vi "Base edit mode.vi"(8 "error in":errorcluster caption="エラー入力（エラーなし）") -> (0 "error out":errorcluster caption="エラー出力", 3 "Base All Composition_out":T1(array[cluster]))   [LabVIEW 2018]
panel:
  in  "R_index":i32
  out "result_number":string
  out "path":path
  in  "N_element":string
  out "filenames":string[](array[string])
  out "stripped path":path
  out "element":string
  in  "insert index":i32
  in  "Base All Composition_edit":T1(array[cluster])
  in  "Base Insert":bool
  in  "New Recipe Creat":bool
  in  "stop":bool
  in  "Edit_index":i32
  in  "Item":T2
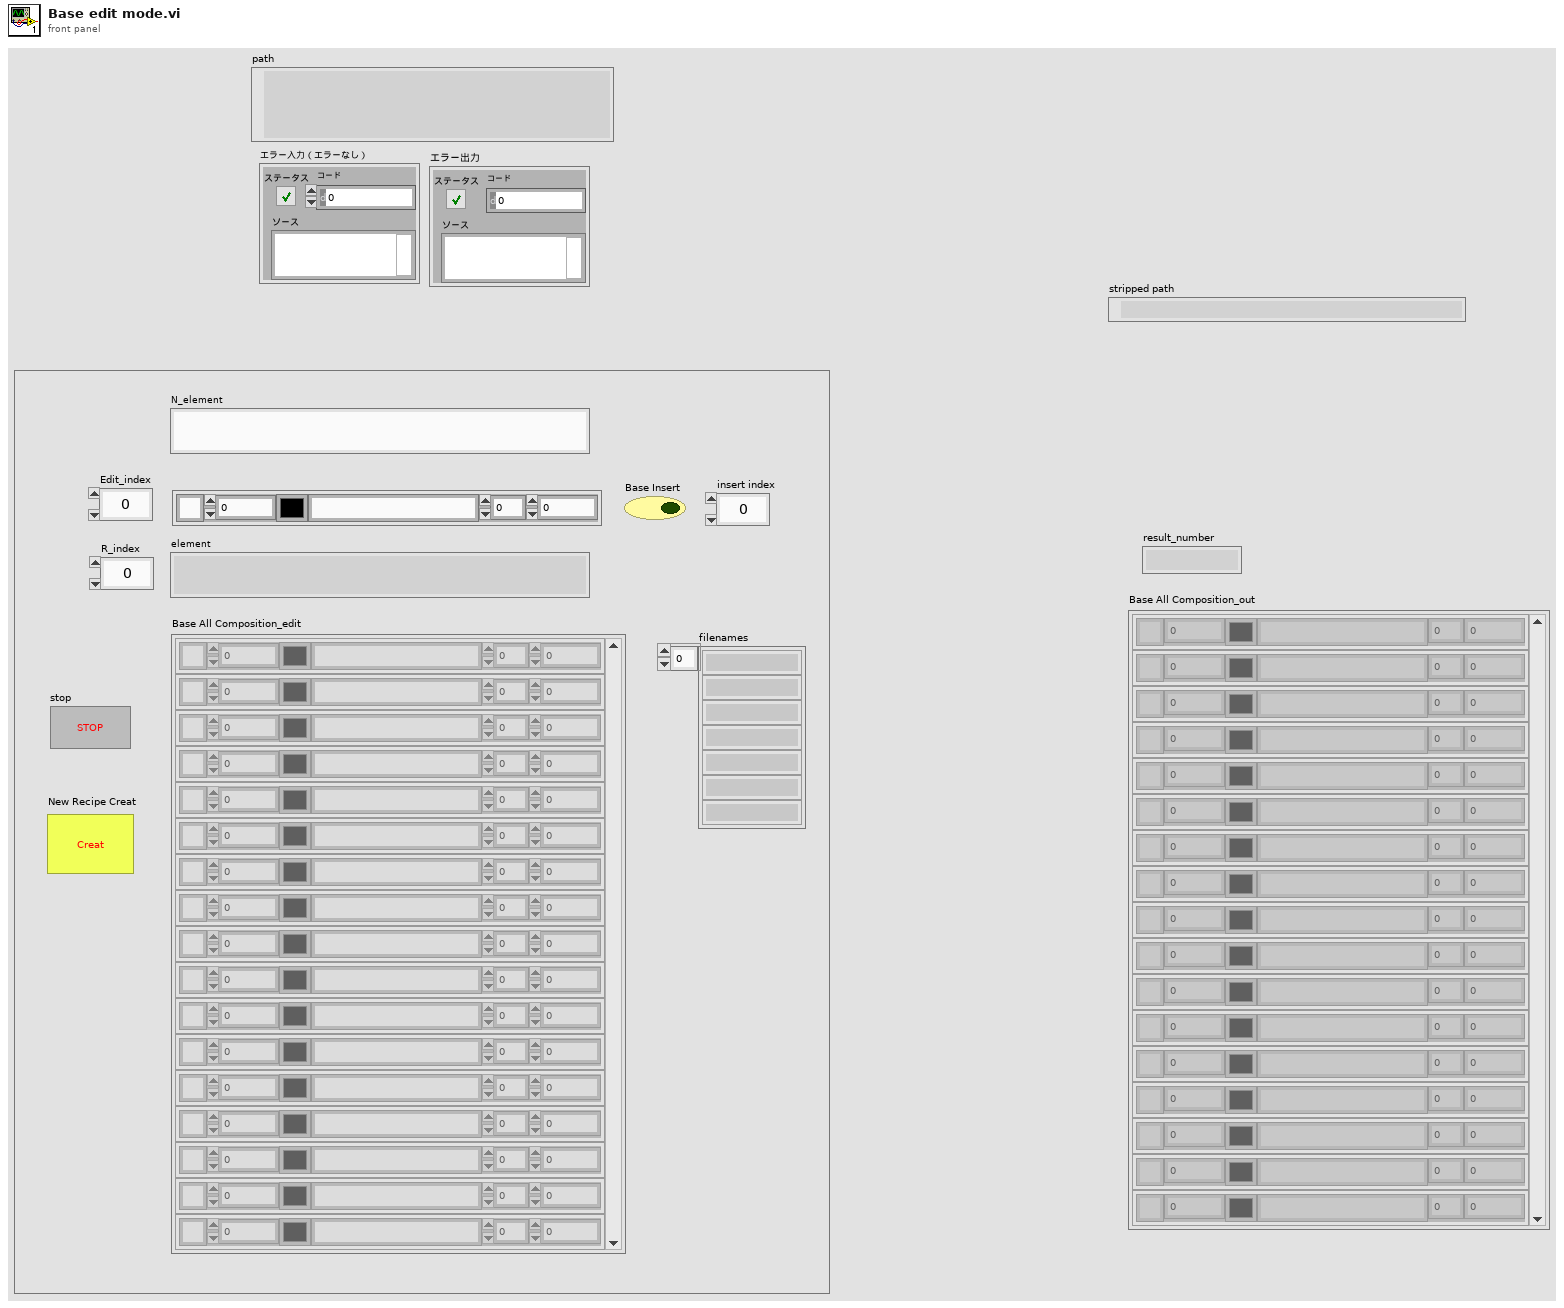
[diagram p1: front panel]
types:
  T1 = cluster{"Name":string, "Value":dbl, "Color":u32, "Name 2":string, "Value 2":dbl, "Value 3":dbl}[]
  T2 = cluster{"Name":string, "Value":dbl, "Color":u32, "Name 2":string, "Value 2":dbl, "Value 3":dbl}
  T3 = enum16{"open", "replace", "create", "open or create", "replace or create", "replace or create with confirmation"}
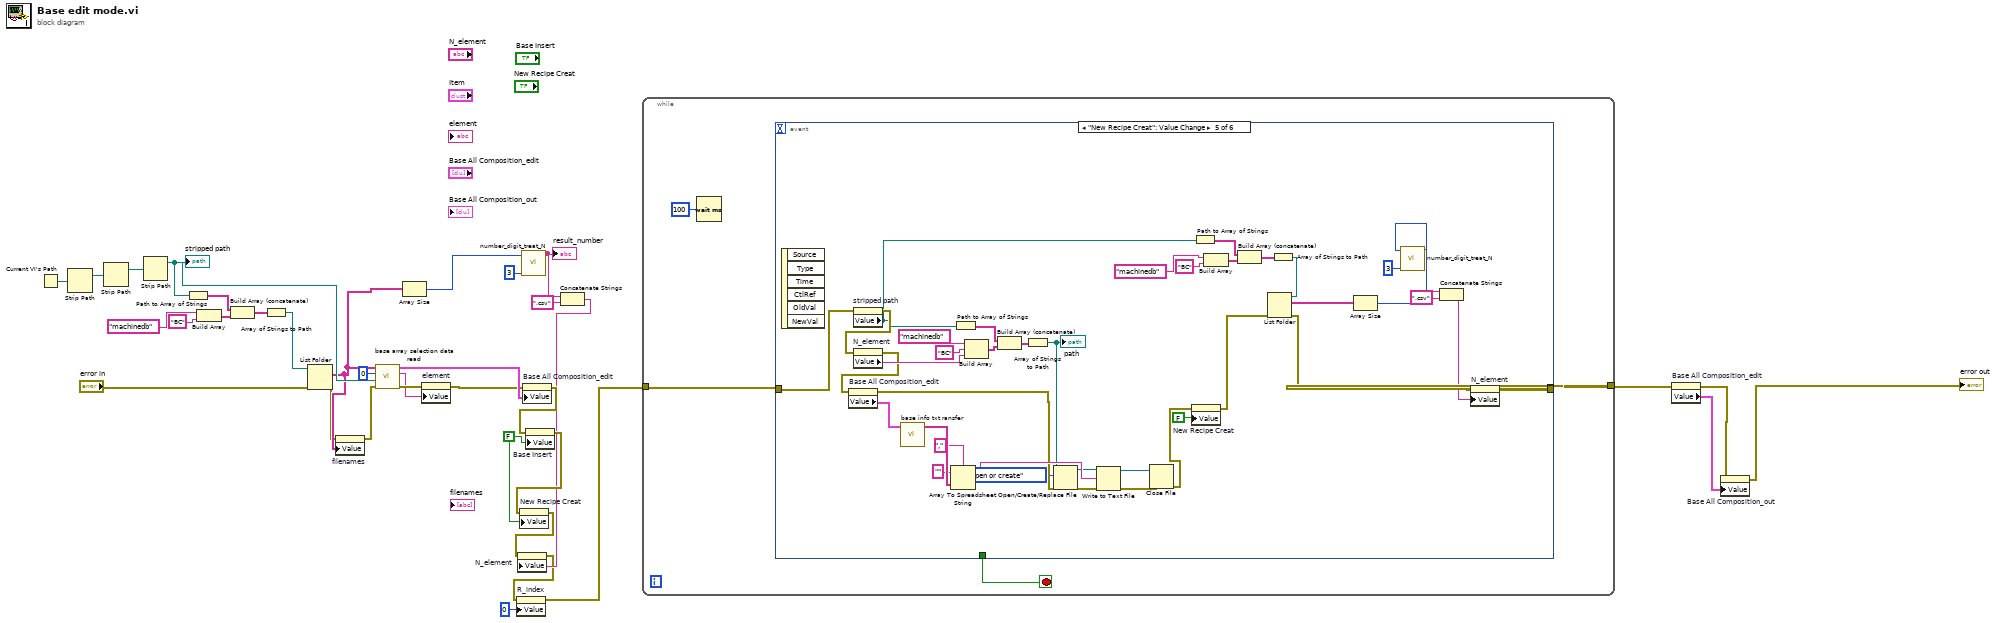
[diagram p0: block diagram]
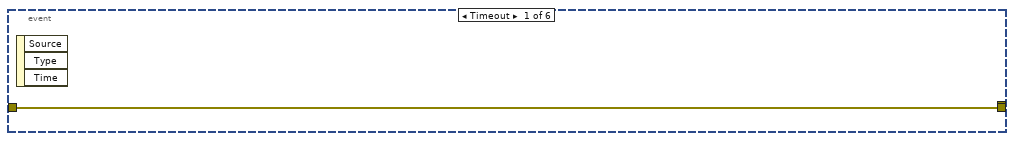
[diagram p2: hidden frame]
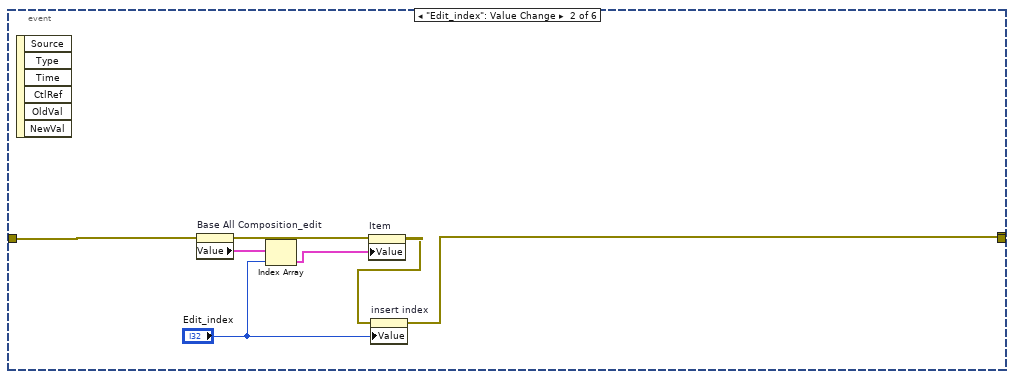
[diagram p3: hidden frame]
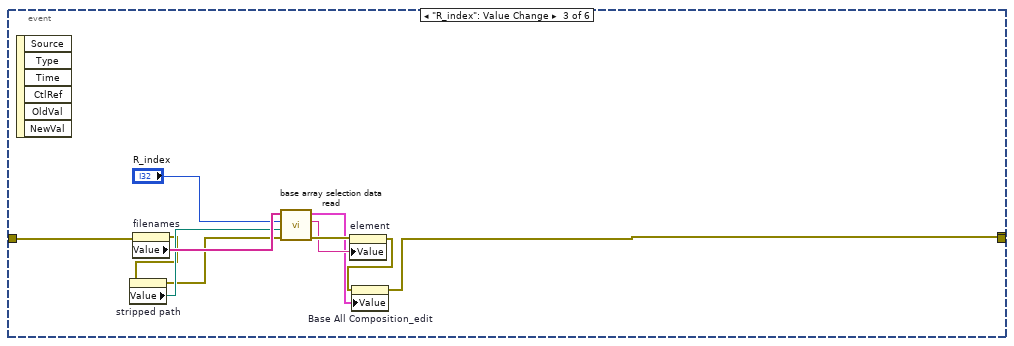
[diagram p4: hidden frame]
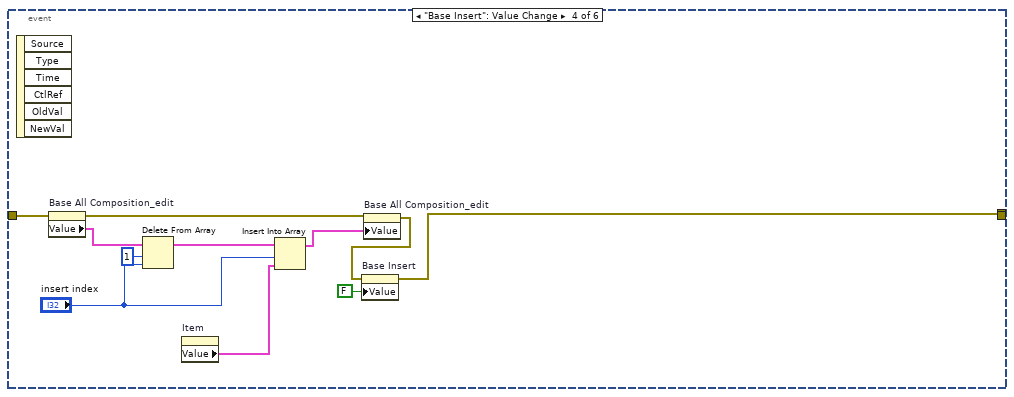
[diagram p5: hidden frame]
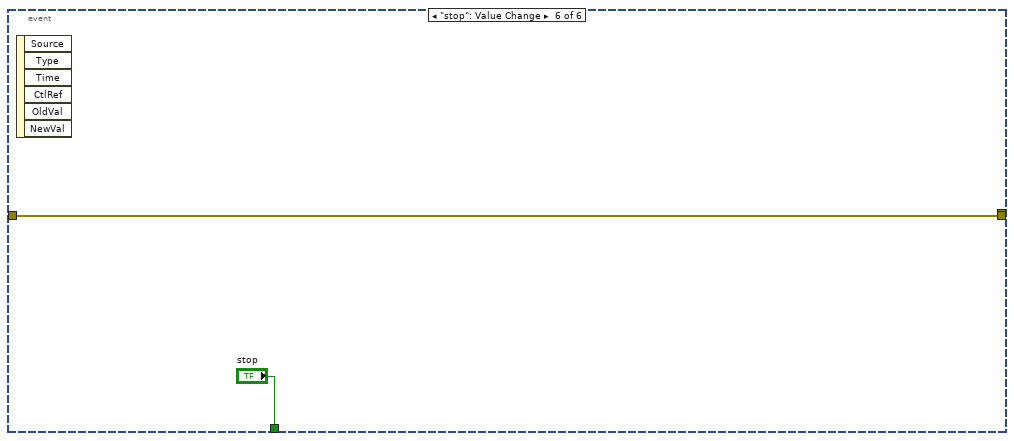
[diagram p6: hidden frame]
diagram:
  w13 = FALSE ("Base Edit")
  n1 = Current VI's Path() -> (path=w31:path)
  n2 = Strip Path(path=w31) -> (stripped path=w30:path)  [unwired: 1 out]
  n3 = Strip Path(path=w30) -> (stripped path=w29:path)  [unwired: 1 out]
  n4 = Strip Path(path=w29) -> (stripped path=w21:path)  [unwired: 1 out]
  "stripped path" <- w21
  n5 = Path to Array of Strings(0:w21) -> (2:w25:string[])  [unwired: 1 out]
  n6 = Build Array("machinedb", "BC") -> (w26:string[])
  n7 = Build Array (concatenate)(w25, w26) -> (w24:string[])
  n8 = Array of Strings to Path(0:w24) -> (2:w23:path)  [unwired: 1 in]
  n9 = List Folder(path=w23, error in="error in") -> (filenames=w3:string[], error out=w2:errorcluster)  [unwired: 2 in, 2 out]
  n10 = property on="filenames" class="Arr (strict)"(error in=w2, "Value"=w3) -> (error out=w1:errorcluster)  [unwired: 1 in, 1 out]
  n11 = call "base array selection data read.vi"("error in"=w1, "stripped path"=w21, "selection"=0, "filenames"=w3) -> ("error out"=w18:errorcluster, "element"=w16:string, "Base All Composition"=w20:T1)  [unwired: 5 in]
  n12 = Array Size(array=w3) -> (size(s)=w11:i32)
  n13 = property on="element" class="Str"(error in=w18, "Value"=w16) -> (error out=w17:errorcluster)  [unwired: 1 in, 1 out]
  n14 = call "number_digit_treat_N.vi"("digit number"=3, "number"=w11) -> ("result_number"=w10:string)  [unwired: 9 in]
  "result_number" <- w10
  n15 = property on="Base All Composition_edit" class="Arr (strict)"(error in=w17, "Value"=w20) -> (error out=w15:errorcluster)  [unwired: 1 in, 1 out]
  n16 = property on="Base Insert" class="Bool (strict)"(error in=w15, "Value"=w13) -> (error out=w14:errorcluster)  [unwired: 1 in, 1 out]
  n17 = property on="New Recipe Creat" class="Bool (strict)"(error in=w14, "Value"=w13) -> (error out=w7:errorcluster)  [unwired: 1 in, 1 out]
  n18 = Concatenate Strings(w10, ".csv" ("string")) -> (w8:string)
  n19 = property on="N_element" class="Str"(error in=w7, "Value"=w8) -> (error out=w5:errorcluster)  [unwired: 1 in, 1 out]
  n20 = property on="R_index" class="DigNum (strict)"(error in=w5, "Value"=0 ("R_index")) -> (error out=w4:errorcluster)  [unwired: 1 in, 1 out]
  n21 = while {
    tunnel: w4 -> [w36]
    tunnel: [w38] -> w34
    stop <- w37 stop-if-true
    n22 = Wait (ms)(milliseconds to wait=u32 100) -> ()  [unwired: 1 out]
    n23 = event shown="[4] \"New Recipe Creat\": Value Change" {
      selector: _ -> [_ _ _ _ _ _]
      dyn-events: _ -> [_ _ _ _ _ _]
      timeout: _ -> [_ _ _ _ _ _]
      tunnel: w36 -> [w40 w46 w56 w69 w102 w109]
      tunnel: [_ w42 w48 w63 w70 w109] -> w38
      tunnel: [_ _ _ _ _ "stop"] -> w37
      tunnel: [w40 _ _ _ _ _] -> _
      event Timeout {
        n24 = event-data() -> ()  [unwired: 1 in, 3 out]
      }
      event "Edit_index": Value Change {
        n25 = event-data() -> ()  [unwired: 1 in, 6 out]
        n26 = property on="Base All Composition_edit" class="Arr (strict)"(error in=w46) -> (error out=w45:errorcluster, "Value"=w47:T1)  [unwired: 1 in, 1 out]
        n27 = Index Array(array=w47, index="Edit_index") -> (element=w44:T2)
        n28 = property on="Item" class="Clust (strict)"(error in=w45, "Value"=w44) -> (error out=w43:errorcluster)  [unwired: 1 in, 1 out]
        n29 = property on="insert index" class="DigNum (strict)"(error in=w43, "Value"="Edit_index") -> (error out=w42:errorcluster)  [unwired: 1 in, 1 out]
      }
      event "R_index": Value Change {
        n30 = event-data() -> ()  [unwired: 1 in, 6 out]
        n31 = property on="filenames" class="Arr (strict)"(error in=w56) -> (error out=w54:errorcluster, "Value"=w58:string[])  [unwired: 1 in, 1 out]
        n32 = property on="stripped path" class="Path"(error in=w54) -> (error out=w53:errorcluster, "Value"=w55:path)  [unwired: 1 in, 1 out]
        n33 = call "base array selection data read.vi"("error in"=w53, "stripped path"=w55, "selection"="R_index", "filenames"=w58) -> ("error out"=w52:errorcluster, "element"=w51:string, "Base All Composition"=w50:T1)  [unwired: 5 in]
        n34 = property on="element" class="Str"(error in=w52, "Value"=w51) -> (error out=w49:errorcluster)  [unwired: 1 in, 1 out]
        n35 = property on="Base All Composition_edit" class="Arr (strict)"(error in=w49, "Value"=w50) -> (error out=w48:errorcluster)  [unwired: 1 in, 1 out]
      }
      event "Base Insert": Value Change {
        n36 = event-data() -> ()  [unwired: 1 in, 6 out]
        n37 = property on="Base All Composition_edit" class="Arr (strict)"(error in=w69) -> (error out=w66:errorcluster, "Value"=w62:T1)  [unwired: 1 in, 1 out]
        n38 = Delete From Array(array=w62, length=1, index="insert index") -> (array with subset deleted=w59:T1)  [unwired: 1 out]
        n39 = property on="Item" class="Clust (strict)"() -> ("Value"=w68:T2)  [unwired: 2 in, 2 out]
        n40 = Insert Into Array(array=w59, index="insert index", new element=w68) -> (w67:T1)
        n41 = property on="Base All Composition_edit" class="Arr (strict)"(error in=w66, "Value"=w67) -> (error out=w64:errorcluster)  [unwired: 1 in, 1 out]
        n42 = property on="Base Insert" class="Bool (strict)"(error in=w64, "Value"=FALSE ("Base Insert")) -> (error out=w63:errorcluster)  [unwired: 1 in, 1 out]
      }
      event "New Recipe Creat": Value Change {
        n43 = event-data() -> ()  [unwired: 1 in, 6 out]
        n44 = property on="stripped path" class="Path"(error in=w102) -> (error out=w101:errorcluster, "Value"=w73:path)  [unwired: 1 in, 1 out]
        n45 = property on="N_element" class="Str"(error in=w101) -> (error out=w99:errorcluster, "Value"=w103:string)  [unwired: 1 in, 1 out]
        n46 = property on="Base All Composition_edit" class="Arr (strict)"(error in=w99) -> (error out=w89:errorcluster, "Value"=w98:T1)  [unwired: 1 in, 1 out]
        n47 = call "base info txt ransfer.vi"("Base All Composition_edit"=w98) -> ("transposed array"=w95:string[][])  [unwired: 10 in]
        n48 = Array To Spreadsheet String(delimiter (Tab)=",", array=w95, 3:"" ("format string")) -> (spreadsheet string=w92:string)
        n49 = Path to Array of Strings(0:w73) -> (2:w105:string[])  [unwired: 1 out]
        n50 = Build Array("machinedb", "BC", w103) -> (w106:string[])
        n51 = Build Array (concatenate)(w105, w106) -> (w104:string[])
        n52 = Array of Strings to Path(0:w104) -> (2:w88:path)  [unwired: 1 in]
        "path" <- w88
        n53 = Open/Create/Replace File(file path (use dialog)=w88, error in=w89, operation (0:open)=T3."open or create") -> (refnum out=w91:refnum<file>, error out=w97:errorcluster)  [unwired: 3 in, 1 out]
        n54 = Write to Text File(file (use dialog)=w91, text=w92, error in=w97) -> (refnum out=w90:refnum<file>, error out=w96:errorcluster)  [unwired: 1 in, 1 out]
        n55 = Close File(refnum=w90, error in=w96) -> (error out=w86:errorcluster)  [unwired: 1 out]
        n56 = property on="New Recipe Creat" class="Bool (strict)"(error in=w86, "Value"=FALSE ("New Recipe Creat")) -> (error out=w74:errorcluster)  [unwired: 1 in, 1 out]
        n57 = Path to Array of Strings(0:w73) -> (2:w80:string[])  [unwired: 1 out]
        n58 = Build Array("machinedb", "BC") -> (w79:string[])
        n59 = Build Array (concatenate)(w80, w79) -> (w81:string[])
        n60 = Array of Strings to Path(0:w81) -> (2:w82:path)  [unwired: 1 in]
        n61 = List Folder(path=w82, error in=w74) -> (filenames=w84:string[], error out=w71:errorcluster)  [unwired: 2 in, 2 out]
        n62 = Array Size(array=w84) -> (size(s)=w85:i32)
        n63 = call "number_digit_treat_N.vi"("digit number"=3, "number"=w85) -> ("result_number"=w83:string)  [unwired: 9 in]
        n64 = Concatenate Strings(w83, ".csv" ("string")) -> (w72:string)
        n65 = property on="N_element" class="Str"(error in=w71, "Value"=w72) -> (error out=w70:errorcluster)  [unwired: 1 in, 1 out]
      }
      event "stop": Value Change {
        n66 = event-data() -> ()  [unwired: 1 in, 6 out]
      }
    }
  }
  n67 = property on="Base All Composition_edit" class="Arr (strict)"(error in=w34) -> (error out=w33:errorcluster, "Value"=w35:T1)  [unwired: 1 in, 1 out]
  n68 = property on="Base All Composition_out" class="Arr (strict)"(error in=w33, "Value"=w35) -> (error out=→"error out":errorcluster)  [unwired: 1 in, 1 out]
